vi "Test Storage Global.vi"(7 "Test Label":string, 9 "Clear (F)":bool, 10 "Set (F)":bool, 11 "VI Call Chain":string[](array[string])) -> (1 "Caller ID":string, 2 "Found/Replaced?":bool, 3 "Unique Test ID":string, 4 "Tests to Register":T1[](array[typedef]))   [LabVIEW 2020, in "Caraya.lvlib" / "Test Assert Factory.lvclass"]
doc: "Keeps track of VIs that have been registered as tests"
uses:
  Test Assert Factory.lvclass
  Test Storage -- cluster.ctl
  Caraya.lvlib
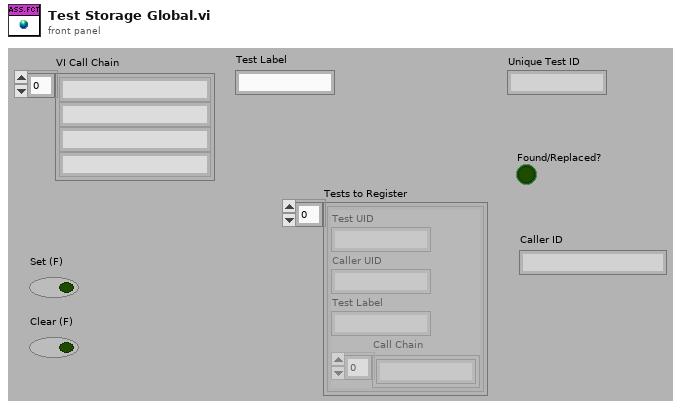
[diagram p1: front panel]
types:
  T1 = typedef "Caraya.lvlib/Test Assert Factory.lvclass/Test Storage -- cluster.ctl" = cluster{"Test UID":string, "Caller UID":string, "Test Label":string, "Call Chain":string[]}
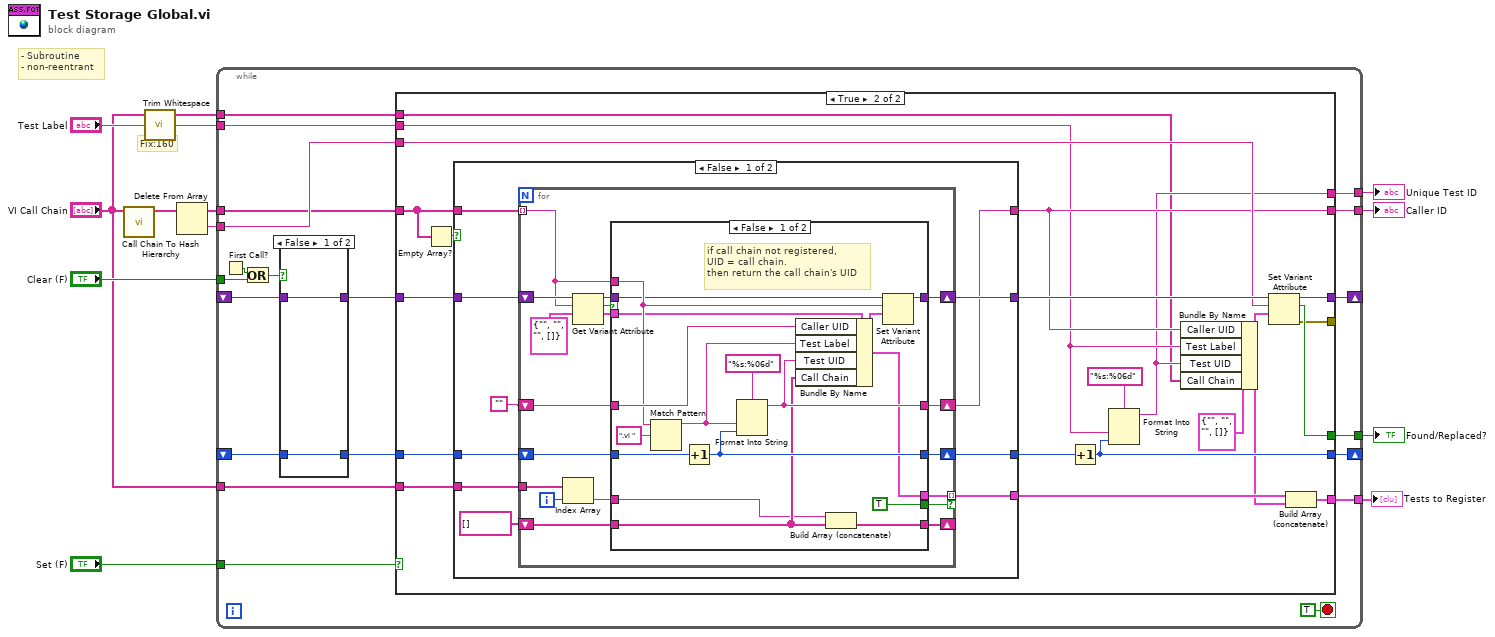
[diagram p0: block diagram]
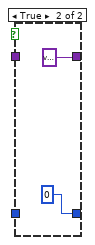
[diagram p2: hidden frame]
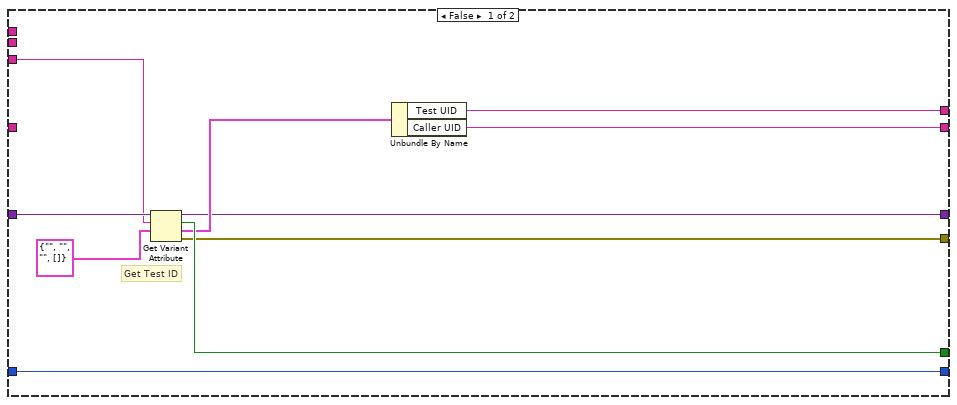
[diagram p3: hidden frame]
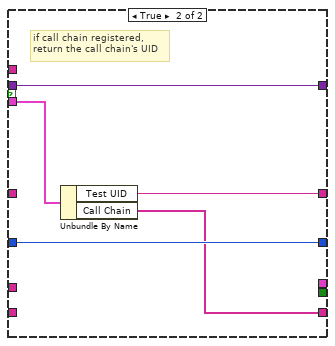
[diagram p4: hidden frame]
diagram:
  # "Fix:160"
  # "- Subroutine\n- non-reentrant"
  n1 = call "Call Chain To Hash Hierarchy.vi"("VI Call Chain"="VI Call Chain") -> ("Flat Hierarchy"=w8:string[])  [unwired: 10 in]
  n2 = call <vilib>:"Trim Whitespace.vi"("string"="Test Label") -> ("trimmed string"=w1:string)  [unwired: 1 in]
  n3 = Delete From Array(array=w8) -> (deleted portion=w6:string, array with subset deleted=w7:string[])  [unwired: 2 in]
  n4 = while {
    tunnel: "Set (F)" -> [w31]
    shift-right: [w28] -> _
    shift-left: _ -> [w30]
    tunnel: [w27] -> w12
    tunnel: "Clear (F)" -> [w17]
    tunnel: w6 -> [w25]
    tunnel: [w24] -> w10
    tunnel: w1 -> [w23]
    shift-right: [w21] -> _
    shift-left: _ -> [w20]
    tunnel: [w19] -> w9
    tunnel: w7 -> [w18]
    tunnel: [w15] -> w3
    tunnel: "VI Call Chain" -> [w14]
    tunnel: "VI Call Chain" -> [w13]
    stop <- TRUE stop-if-true
    n5 = First Call?() -> (First Call?: T/F=w26:bool)
    n6 = Or(x=w26, y=w17) -> (x .or. y?=w16:bool)
    n7 = case shown="False" w16 {
      tunnel: w30 -> [w34 _]
      tunnel: [w34 variant ("variant")] -> w29
      tunnel: [w33 u32 0] -> w22
      tunnel: w20 -> [w33 _]
      frame False {
      }
      frame True {
      }
    }
    n8 = case shown="True" w31 {
      tunnel: w29 -> [w46 w64]
      tunnel: [w38 w61] -> w28
      tunnel: [w45 w67] -> w27
      tunnel: w25 -> [w43 w55]
      tunnel: [w41 w52] -> w24
      tunnel: w23 -> [_ w53]
      tunnel: w22 -> [w44 w58]
      tunnel: [w44 w66] -> w21
      tunnel: [w40 w54] -> w19
      tunnel: [w37 w60] -> _
      tunnel: w18 -> [_ w62]
      tunnel: [_ w49] -> w15
      tunnel: w14 -> [_ w48]
      tunnel: w13 -> [_ w47]
      frame False {
        # "Get Test ID"
        n9 = Get Variant Attribute(Variant=w46, name=w43, default value (empty Variant)=T1 {"Test UID"="", "Caller UID"="", "Test Label"="", "Call Chain"=[]} ("Test")) -> (duplicate Variant=w38:variant, found=w45:bool, value=w42:T1, error out=w37:errorcluster)  [unwired: 1 in]
        n10 = Unbundle By Name(w42) -> ("Test UID"=w41:string, "Caller UID"=w40:string)
      }
      frame True {
        n11 = Empty Array?(array=w62) -> (empty?=w59:bool)
        n12 = case shown="False" w59 {
          tunnel: w64 -> [w77 w118]
          tunnel: [w76 w118] -> w63
          tunnel: [w73 _] -> w54
          tunnel: w62 -> [w75 _]
          tunnel: w58 -> [w72 w117]
          tunnel: [w71 w117] -> w57
          tunnel: [w70 _] -> w51
          tunnel: w47 -> [w69 _]
          frame False {
            n13 = for {
              shift-right: [w95] -> w76
              shift-left: w77 -> [w94]
              tunnel: w75 -> [w92] mode=indexing
              shift-right: [w89] -> w73
              shift-left: "" -> [w88]
              shift-right: [w86] -> w71
              shift-left: w72 -> [w87]
              tunnel: [w84] -> w70 mode=indexing if=w83
              tunnel: w69 -> [w82]
              shift-right: [w78] -> _
              shift-left: string[] [] ("VI Call Chain") -> [w80]
              i -> [w81]
              n14 = Index Array(array=w82, index=w81) -> (element=w79:string)
              n15 = Get Variant Attribute(Variant=w94, name=w92, default value (empty Variant)=T1 {"Test UID"="", "Caller UID"="", "Test Label"="", "Call Chain"=[]} ("Test")) -> (duplicate Variant=w93:variant, found=w91:bool, value=w90:T1)  [unwired: 1 in, 1 out]
              n16 = case shown="False" w91 {
                tunnel: [w111 w116] -> w95
                tunnel: w93 -> [w103 w116]
                tunnel: w92 -> [w106 _]
                tunnel: w90 -> [w104 w113]
                tunnel: [w102 w114] -> w89
                tunnel: w88 -> [w107 _]
                tunnel: w87 -> [w109 w115]
                tunnel: [w108 w115] -> w86
                tunnel: [w100 _] -> w84
                tunnel: [TRUE _] -> w83
                tunnel: w80 -> [w98 _]
                tunnel: w79 -> [w97 _]
                tunnel: [w96 w112] -> w78
                frame False {
                  # "if call chain not registered, \nUID = call chain.\nthen return the call chain's UID"
                  n17 = Match Pattern(string=w106, regular expression=".vi ") -> (before substring=w101:string)  [unwired: 1 in, 3 out]
                  n18 = Increment(x=w109) -> (x+1=w108:u32)
                  n19 = Format Into String(format string="%s:%06d", w101, w108) -> (resulting string=w102:string)  [unwired: 2 in, 1 out]
                  n20 = Bundle By Name(cluster=w104, "Caller UID"=w107, "Test Label"=w101, "Test UID"=w102, "Call Chain"=w98) -> (w100:T1)
                  n21 = Build Array (concatenate)(w97, w98) -> (w96:string[])
                  n22 = Set Variant Attribute(Variant=w103, name=w106, value=w100) -> (Variant out=w111:variant)  [unwired: 1 in, 2 out]
                }
                frame True {
                  # "if call chain registered, \nreturn the call chain's UID"
                  n23 = Unbundle By Name(w113) -> ("Test UID"=w114:string, "Call Chain"=w112:string[])
                }
              }
            }
          }
          frame True {
          }
        }
        n24 = Increment(x=w57) -> (x+1=w66:u32)
        n25 = Format Into String(format string="%s:%06d", w53, w66) -> (resulting string=w52:string)  [unwired: 2 in, 1 out]
        n26 = Bundle By Name(cluster=T1 {"Test UID"="", "Caller UID"="", "Test Label"="", "Call Chain"=[]} ("Test"), "Caller UID"=w54, "Test Label"=w53, "Test UID"=w52, "Call Chain"=w48) -> (w50:T1)
        n27 = Set Variant Attribute(Variant=w63, name=w55, value=w50) -> (Variant out=w61:variant, replaced=w67:bool, error out=w60:errorcluster)  [unwired: 1 in]
        n28 = Build Array (concatenate)(w51, w50) -> (w49:T1[])
      }
    }
  }
  "Found/Replaced?" <- w12
  "Unique Test ID" <- w10
  "Caller ID" <- w9
  "Tests to Register" <- w3
